vi "VIH HelpGen - FILE - Check File Path (Buffered).vi"(7 "cmd (get)":enum16{"Init", "get"}(ring)=enum."get", 10 "Force Update (T)":bool=TRUE, 11 "File Path":path) -> (2 "Good path":bool, 3 "dup File Path":path)   [LabVIEW 2014]
doc: "::: VI Helpeks :::\nCopyright (c) 2000-2026 Konstantin Shifershteyn. All rights reserved."
panel:
  # "VI Helpeks\nCopyright (c) 2012-2026 Konstantin Shifershteyn"
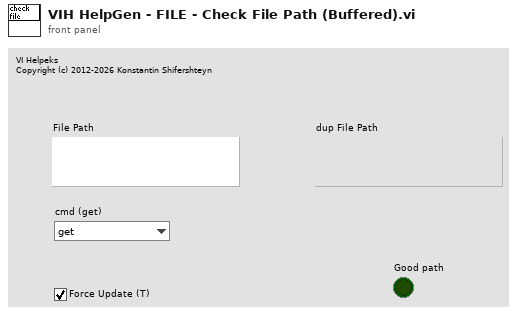
[diagram p1: front panel]
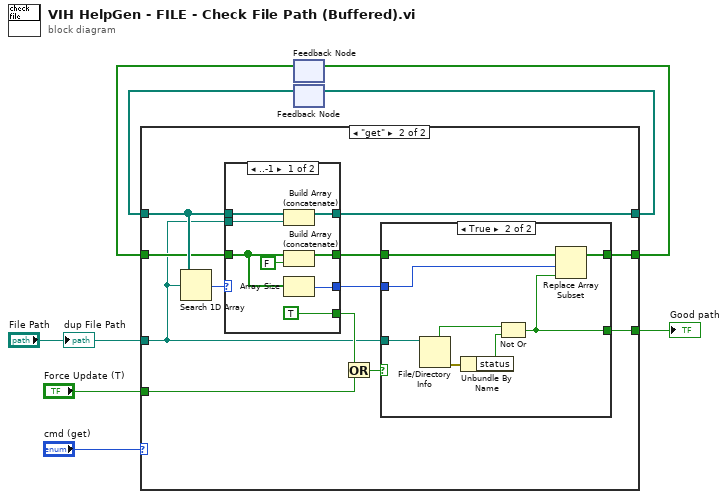
[diagram p0: block diagram]
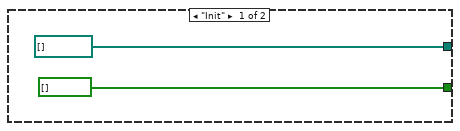
[diagram p2: hidden frame]
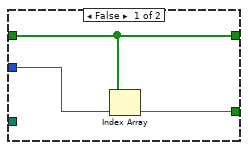
[diagram p3: hidden frame]
diagram:
  n1 = feedback #1() -> (w4:bool[])  [unwired: 1 in]
  n2 = feedback #2() -> (w6:path[])  [unwired: 1 in]
  n3 = case shown="\"get\"" "cmd (get)" {
    tunnel: [path[] [] w19] -> w7
    tunnel: w6 -> [_ w21]
    tunnel: [bool[] [] w12] -> w5
    tunnel: w4 -> [_ w20]
    tunnel: "File Path" -> [_ w15]
    tunnel: "Force Update (T)" -> [_ w17]
    tunnel: [_ w11] -> w2
    frame "Init" {
    }
    frame "get" {
      n4 = Search 1D Array(1D array=w21, element=w15) -> (index of element=w22:i32)  [unwired: 1 in]
      n5 = case shown="..-1" w22 {
        selector: w22 -> [_ w42]
        tunnel: [w40 w44] -> w19
        tunnel: w21 -> [w41 w44]
        tunnel: [w39 w43] -> w13
        tunnel: w20 -> [w34 w43]
        tunnel: w15 -> [w38 _]
        tunnel: [TRUE _] -> w18
        tunnel: [w35 w42] -> w14
        frame ..-1 {
          n6 = Build Array (concatenate)(w41, w38) -> (w40:path[])
          n7 = Build Array (concatenate)(w34, FALSE) -> (w39:bool[])
          n8 = Array Size(array=w34) -> (size(s)=w35:i32)
        }
        frame 0.. {
        }
      }
      n9 = Or(x=w18, y=w17) -> (x .or. y?=w16:bool)
      n10 = case shown="True" w16 {
        tunnel: w15 -> [_ w30]
        tunnel: w14 -> [w23 w27]
        tunnel: w13 -> [w25 w29]
        tunnel: [w25 w28] -> w12
        tunnel: [w24 w26] -> w11
        frame False {
          n11 = Index Array(array=w25, index=w23) -> (element=w24:bool)
        }
        frame True {
          n12 = File/Directory Info(path=w30) -> (directory=w32:bool, error out=w31:errorcluster)  [unwired: 1 in, 5 out]
          n13 = Unbundle By Name(w31) -> ("status"=w33:bool)
          n14 = Not Or(1:w33, 2:w32) -> (0:w26:bool)
          n15 = Replace Array Subset(array=w29, new element=w26, index=w27) -> (w28:bool[])
        }
      }
    }
  }
  "Good path" <- w2
  n16 = feedback-in #1(w5) -> ()
  n17 = feedback-in #2(w7) -> ()
  "dup File Path" <- "File Path"
